vi "DSS-Tests-water_perm_case.vi"(8 "error in":errorcluster, 9 "frequency":dbl[](array[numeric]), 10 "temperature":dbl=22.5, 11 "golden name":string) -> (0 "error out":errorcluster, 2 "message":string, 3 "pass":bool)   [LabVIEW 2020, in "DSS-Tests.lvlib"]
doc: "One golden case of RDC-water-generate_perm_from_freq: runs it at a temperature over a frequency array and checks Complex Perm, Real Perm, Imag Perm, Complex perm and used temp, flattened, against the named golden file."
uses:
  DSS-Tests.lvlib
  Computation/RDC-Reflection_Data_Computation.lvlib
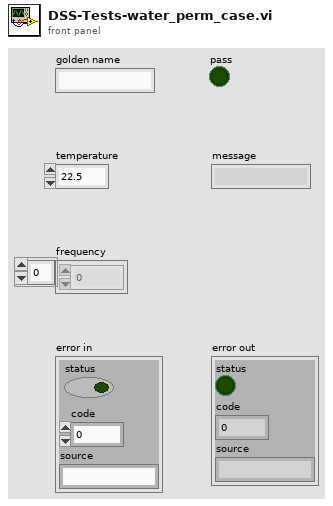
[diagram p1: front panel]
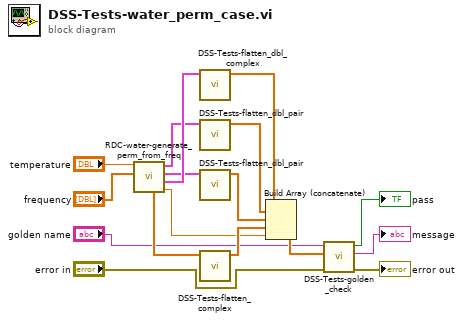
[diagram p0: block diagram]
diagram:
  n1 = call "RDC-water-generate_perm_from_freq.vi"("Frequency"="frequency", "water Temp (25C) [10-40C]"="temperature") -> ("used temp"=w9:dbl, "Complex Perm"=w7:cluster{dbl[], cdb[]}, "Imag Perm"=w6:cluster{dbl[], dbl[]}, "Real Perm"=w5:cluster{dbl[], dbl[]}, "Complex perm"=w8:cdb[])  [unwired: 5 in]
  n2 = call "DSS-Tests-flatten_dbl_complex.vi"("pair"=w7) -> ("flat"=w10:dbl[])  [unwired: 10 in]
  n3 = call "DSS-Tests-flatten_dbl_pair.vi"("pair"=w5) -> ("flat"=w11:dbl[])  [unwired: 10 in]
  n4 = call "DSS-Tests-flatten_dbl_pair.vi"("pair"=w6) -> ("flat"=w12:dbl[])  [unwired: 10 in]
  n5 = call "DSS-Tests-flatten_complex.vi"("values"=w8) -> ("flat"=w13:dbl[])  [unwired: 10 in]
  n6 = Build Array (concatenate)(w10, w11, w12, w13, w9) -> (w14:dbl[])
  n7 = call "DSS-Tests-golden_check.vi"("error in"="error in", "actual"=w14, "golden name"="golden name") -> ("error out"=→"error out":errorcluster, "message"=→"message":string, "pass"=→"pass":bool)  [unwired: 6 in]
